vi "Post-Build Action.vi"(5 "Files Generated by Build":path[](array[path]), 6 "Top Level/Always Included VIs":path[](array[path]), 7 "Destination Path":path, 8 "error in (no error)":errorcluster, 9 "Target Name":string, 10 "Build Specification Name":string, 11 "Project Path":path) -> (0 "error out":errorcluster)   [LabVIEW 2027, in "Build VIs.lvlib"]
uses:
  Build VIs.lvlib
  <vilib>/Utility/sysdir.llb/System Directory Type.ctl
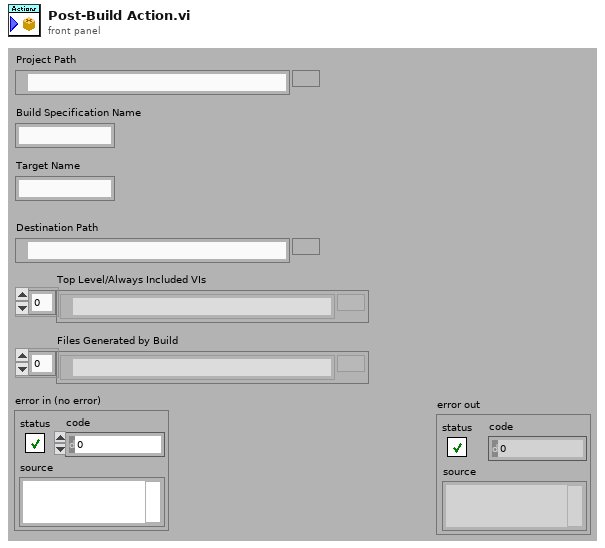
[diagram p1: front panel]
types:
  T1 = typedef "System Directory Type.ctl" = i32
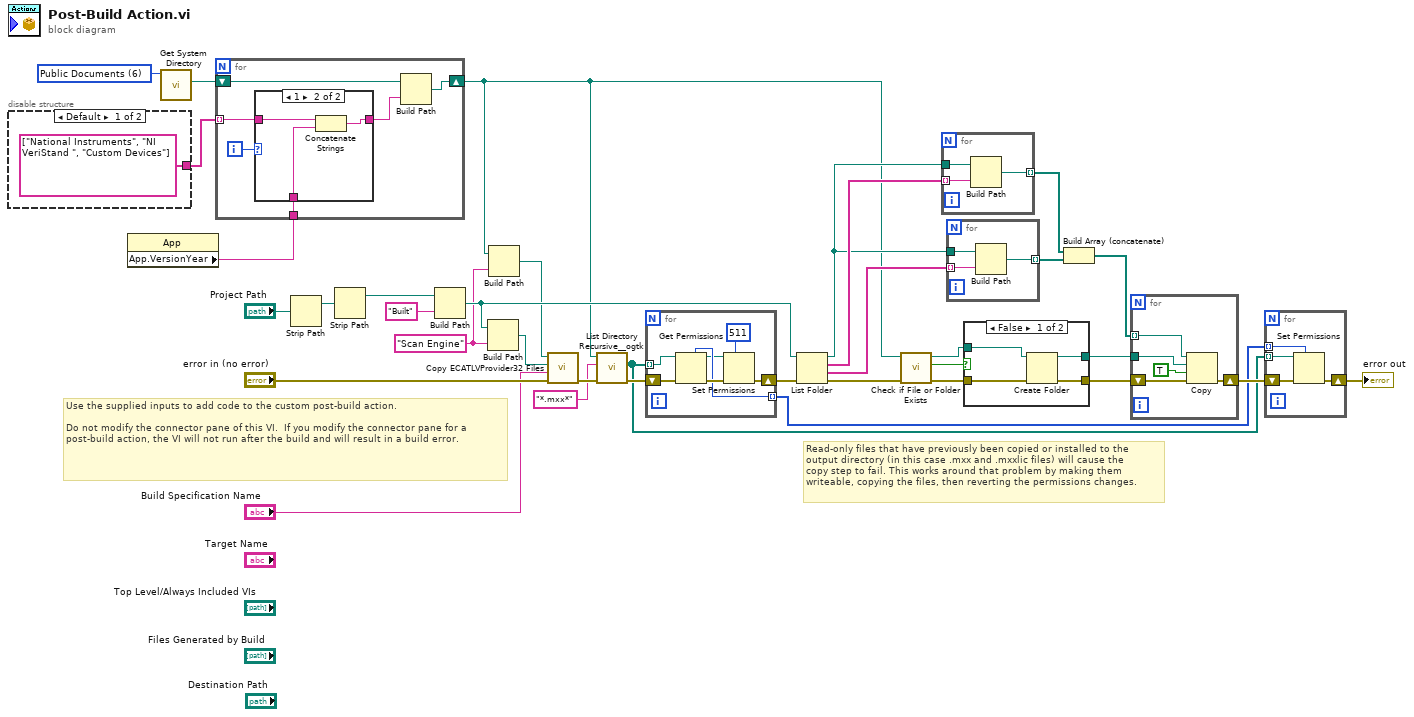
[diagram p0: block diagram]
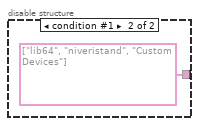
[diagram p2: hidden frame]
diagram:
  w13 = "Scan Engine" ("name or relative path")
  w18 = T1 6 items=["User Home"=0, "User Desktop"=1, "User Documents"=2, "User Application Data"=3, "User Preferences"=4, "User Temporary"=5, "Public Documents"=6, "Public Application Data"=7, "Public Preferences"=8, "Public Cache"=13, "System Core Libraries"=9, "System Installed Libraries"=10, "Application Files"=11, "Boot Volume Root"=12] ("system directory type")
  # "Read-only files that have previously been copied or installed to the\noutput directory (in this case .mxx and .mxxlic files) will cause the\ncopy step to fail. This works around that problem by making them\nwriteable, copying the files, then reverting the permissions changes."
  # "Use the supplied inputs to add code to the custom post-build action.\n\nDo not modify the connector pane of this VI.  If you modify the connector pane for a post-build action, the VI will not run after the build and will result in a build error."
  n1 = disable-structure shown="Default" {
    disable-tunnel: [string[] ["National Instruments", "NI VeriStand ", "Custom Devices"] string[] ["lib64", "niveristand", "Custom Devices"]] -> w16
    frame condition #0 (active) {
    }
    frame condition #1 {
    }
  }
  n2 = property class="App"() -> ("App.VersionYear"=w15:string)  [unwired: 2 in, 2 out]
  n3 = call <vilib>:"Get System Directory.vi"("system directory type"=w18) -> ("system directory"=w17:path)  [unwired: 10 in]
  n4 = for {
    shift-right: [w42] -> w9
    shift-left: w17 -> [w43]
    tunnel: w16 -> [w39] mode=indexing
    tunnel: w15 -> [w38]
    i -> [w41]
    n5 = case shown="1" w41 {
      tunnel: [w44 w46] -> w40
      tunnel: w39 -> [w44 w47]
      tunnel: w38 -> [_ w45]
      frame Default {
      }
      frame 1 {
        n6 = Concatenate Strings(w47, w45) -> (w46:string)
      }
    }
    n7 = Build Path(base path=w43, name or relative path=w40) -> (appended path=w42:path)
  }
  n8 = Strip Path(path="Project Path") -> (stripped path=w21:path)  [unwired: 1 out]
  n9 = Strip Path(path=w21) -> (stripped path=w31:path)  [unwired: 1 out]
  n10 = Build Path(base path=w31, name or relative path="Built") -> (appended path=w14:path)
  n11 = Build Path(base path=w14, name or relative path=w13) -> (appended path=w11:path)
  n12 = Build Path(base path=w9, name or relative path=w13) -> (appended path=w12:path)
  n13 = call "Copy ECATLVProvider32 Files.vi"("error in"="error in (no error)", "Build Specification Name"="Build Specification Name", "Source Path"=w11, "Destination Path"=w12) -> ("error out"=w10:errorcluster)  [unwired: 7 in]
  n14 = call <userlib>:"List Directory Recursive__ogtk.vi"("error in (no error)"=w10, "pattern"="*.mxx*", "Path"=w9) -> ("error out"=w7:errorcluster, "file paths"=w3:path[])  [unwired: 5 in, 2 out]
  n15 = for {
    shift-right: [w53] -> w6
    shift-left: w7 -> [w52]
    tunnel: w3 -> [w50] mode=indexing
    tunnel: [w49] -> w2 mode=indexing
    n16 = Get Permissions(8:w52, 11:w50) -> (0:w51:errorcluster, 3:w48:path, 5:w49:i16)  [unwired: 2 out]
    n17 = Set Permissions(7:i16 511 ("permissions"), 8:w51, 11:w48) -> (0:w53:errorcluster)  [unwired: 2 in, 1 out]
  }
  n18 = List Folder(path=w14, error in=w6) -> (path out=w23:path, filenames=w35:string[], folder names=w24:string[], error out=w19:errorcluster)  [unwired: 2 in]
  n19 = call <vilib>:"Check if File or Folder Exists.vi"("error in (no error)"=w19, "path"=w9) -> ("error out"=w27:errorcluster, "file or folder exists?"=w29:bool, "dup path"=w28:path)  [unwired: 7 in]
  n20 = for {
    tunnel: w35 -> [w56] mode=indexing
    tunnel: w23 -> [w57]
    tunnel: [w55] -> w34 mode=indexing
    n21 = Build Path(base path=w57, name or relative path=w56) -> (appended path=w55:path)
  }
  n22 = for {
    tunnel: w24 -> [w59] mode=indexing
    tunnel: w23 -> [w60]
    tunnel: [w58] -> w22 mode=indexing
    n23 = Build Path(base path=w60, name or relative path=w59) -> (appended path=w58:path)
  }
  n24 = case shown="False" w29 {
    tunnel: w28 -> [w64 w66]
    tunnel: w27 -> [w63 w65]
    tunnel: [w62 w66] -> w26
    tunnel: [w61 w65] -> w25
    frame False {
      n25 = Create Folder(path (use dialog)=w64, error in=w63) -> (created path=w62:path, error out=w61:errorcluster)  [unwired: 1 in, 1 out]
    }
    frame True {
    }
  }
  n26 = Build Array (concatenate)(w34, w22) -> (w33:path[])
  n27 = for {
    tunnel: w33 -> [w68] mode=indexing
    shift-right: [w69] -> w5
    shift-left: w25 -> [w70]
    tunnel: w26 -> [w67]
    n28 = Copy(8:w70, 9:TRUE ("overwrite (F)"), 10:w67, 11:w68) -> (0:w69:errorcluster)  [unwired: 1 in, 2 out]
  }
  n29 = for {
    shift-right: [w75] -> w4
    shift-left: w5 -> [w74]
    tunnel: w3 -> [w73] mode=indexing
    tunnel: w2 -> [w72] mode=indexing
    n30 = Set Permissions(7:w72, 8:w74, 11:w73) -> (0:w75:errorcluster)  [unwired: 2 in, 1 out]
  }
  "error out" <- w4
